vi "Manual UI.vi"(11 "Bus Access":refnum<class "Bus_Access.lvclass">[](array[class])) -> ()   [LabVIEW 2021]
uses:
  <vilib>/TSA/Omni-Bus/Omni-Bus/Bus Access/Bus_Access.lvclass
  <vilib>/TSA/Omni-Bus/Omni-Bus/Omni_Bus.lvclass
  <vilib>/TSA/Omni-Bus/Omni-Bus/Support/Write/Write DBL.vi
  <vilib>/TSA/Abstract Data Classes/Abs_Types/Double Float/Abs_Double Float.lvclass
  C:/Program Files (x86)/National Instruments/LabVIEW 2021/vi.lib/TSA/Abstract Data Classes/Abs_Types/Type/Abs_Type.lvclass
  <vilib>/TSA/Omni-Bus/Omni-Bus/Support/FindVar.vi
panel:
  in  "SImulated Temp":dbl(slide) scale=20.0..80.0
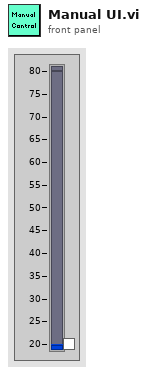
[diagram p1: front panel]
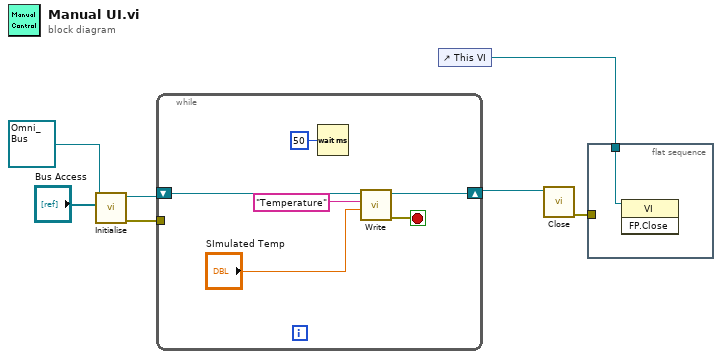
[diagram p0: block diagram]
diagram:
  n1 = call-dynamic "Initialise.vi"("Bus Access"="Bus Access", "Var Bus in"=refnum<class "Omni_Bus.lvclass"> refnum) -> ("error out"=w3:errorcluster, "Var Bus out"=w6:refnum<class "Omni_Bus.lvclass">)  [unwired: 8 in]
  n2 = while {
    shift-right: [w10] -> w5
    shift-left: w6 -> [w11]
    tunnel: w3 -> [_]
    stop <- w9 stop-if-true
    n3 = Wait (ms)(milliseconds to wait=u32 50) -> ()  [unwired: 1 out]
    n4 = call-poly <vilib>:"Write.vi"("Numeric"="SImulated Temp", "Tag"="Temperature", "Omni_Bus in"=w11) -> ("error out"=w9:errorcluster, "Omni_Bus out"=w10:refnum<class "Omni_Bus.lvclass">)  [unwired: 7 in]
  }
  n5 = control-ref of="This VI"() -> (w2:refnum<vi>)
  n6 = call-dynamic "Close.vi"("Data in"=w5) -> ("error out"=w1:errorcluster)  [unwired: 9 in, 1 out]
  n7 = flat-sequence {
    tunnel: w2 -> [w14]
    tunnel: w1 -> [_]
    frame #0 {
      n8 = invoke class="VI" method="FP.Close"(reference=w14) -> ()  [unwired: 2 in, 3 out]
    }
  }
